vi "XML_to_Variant.vi"(8 "error in (no error)":errorcluster, 11 "arg1":string) -> (0 "error out":errorcluster, 3 "Variant":variant)   [LabVIEW 2020]
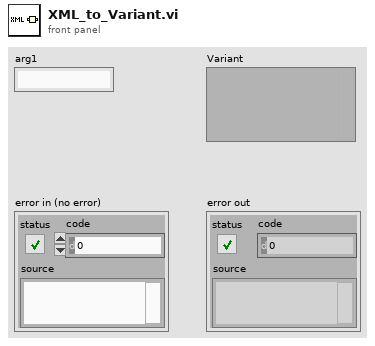
[diagram p1: front panel]
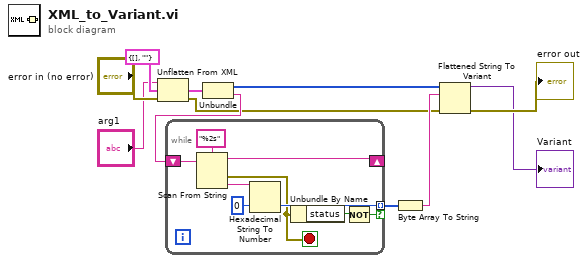
[diagram p0: block diagram]
diagram:
  n1 = Unflatten From XML(xml string="arg1", type=cluster{"type string":i16[], string} {"type string"=[], ""} ("output cluster"), error in (no error)="error in (no error)") -> (value=w4:cluster{"type string":i16[], string}, error out=w7:errorcluster)
  n2 = Unbundle(w4) -> ("type string"=w5:i16[], w10:string)
  n3 = while {
    shift-right: [w20] -> _
    shift-left: w10 -> [w19]
    tunnel: [w16] -> w9 mode=indexing if=w13
    stop <- w15 stop-if-true
    n4 = Scan From String(format string="%2s", input string=w19) -> (remaining string=w20:string, error out=w15:errorcluster, output 1=w17:string)  [unwired: 3 in, 1 out]
    n5 = Hexadecimal String To Number(string=w17, default (0uL)=u8 0) -> (number=w16:u8)  [unwired: 1 in, 1 out]
    n6 = Unbundle By Name(w15) -> ("status"=w14:bool)
    n7 = Not(x=w14) -> (.not. x?=w13:bool)
  }
  n8 = Byte Array To String(unsigned byte array=w9) -> (string=w11:string)
  n9 = Flattened String To Variant(4:w7, 6:w11, 7:w5) -> (0:→"error out":errorcluster, 3:→"Variant":variant)
